vi "LabApp - Run Top-Level VIs.vi"(6 "error in (no error)":errorcluster) -> (0 "error out":errorcluster)   [LabVIEW 2021]
doc: "::: CalcExpress Toolkit :::\nCopyright (c) 2000-2026 Konstantin Shifershteyn. All rights reserved."
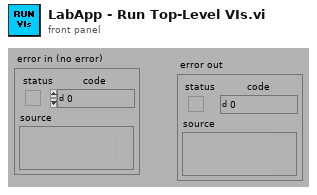
[diagram p1: front panel]
types:
  T1 = enum32{"Bad", "Idle", "Run top level", "Running"}
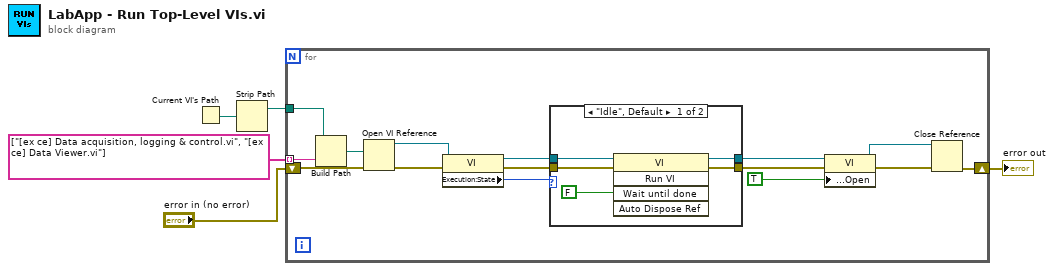
[diagram p0: block diagram]
diagram:
  n1 = Current VI's Path() -> (path=w4:path)
  n2 = Strip Path(path=w4) -> (stripped path=w3:path)  [unwired: 1 out]
  n3 = for {
    tunnel: string[] ["[ex ce] Data acquisition, logging & control.vi", "[ex ce] Data Viewer.vi"] -> [w20] mode=indexing
    tunnel: w3 -> [w19]
    shift-right: [w7] -> w1
    shift-left: "error in (no error)" -> [w6]
    n4 = Build Path(base path=w19, name or relative path=w20) -> (appended path=w18:path)
    n5 = Open VI Reference(vi path=w18, error in (no error)=w6) -> (vi reference=w16:refnum<vi>, error out=w17:errorcluster)  [unwired: 4 in]
    n6 = property class="VI"(reference=w16, error in=w17) -> (reference out=w13:refnum<vi>, error out=w14:errorcluster, "Execution:State"=w15:T1)
    n7 = case shown="\"Idle\", Default" w15 {
      tunnel: w14 -> [w25 w26]
      tunnel: w13 -> [w24 w27]
      tunnel: [w22 w27] -> w12
      tunnel: [w21 w26] -> w11
      frame "Idle", Default {
        n8 = invoke class="VI" method="Run VI"(reference=w24, error in=w25, "Wait until done"=FALSE) -> (reference out=w22:refnum<vi>, error out=w21:errorcluster)  [unwired: 2 in, 3 out]
      }
      frame "Run top level" {
      }
    }
    n9 = property class="VI"(reference=w12, error in=w11, "Front Panel Window:Open"=TRUE ("Front Panel.Open")) -> (reference out=w8:refnum<vi>, error out=w9:errorcluster)
    n10 = Close Reference(reference=w8, error in (no error)=w9) -> (error out=w7:errorcluster)
  }
  "error out" <- w1
